vi "Module Loop.vi"(8 "error in (no error)":errorcluster, 11 "Data Processor Module in":refnum<class "Data Processor Module.lvclass">) -> (0 "error out":errorcluster, 3 "Data Processor Module out":refnum<class "Data Processor Module.lvclass">)   [LabVIEW 2020, in "VolatusData.lvlib" / "Data Processor Module.lvclass"]
uses:
  Data Processor Module.lvclass
  C:/dev/lv20CE/relink/lv-volatus/Volatus/Module/Module.lvclass
  Volatus/Module/Module.lvclass
  Data Processor Module.lvclass/Data Processor Module.ctl
  New Data.ctl
  Volatus/Module/Module.lvclass/Module.ctl
  <vilib>/Utility/error.llb/Error Cluster From Error Code.vi
  VolatusData.lvlib
panel:
  out "Parent":string
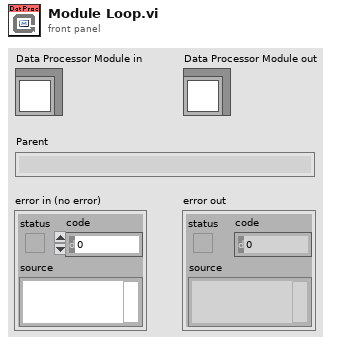
[diagram p1: front panel]
types:
  T1 = enum32{"Invalid", "Standard", "Closed", "Hidden", "Minimized", "Maximized"}
  T2 = typedef "VolatusData.lvlib/New Data.ctl" = cluster{"Channels":waveform(dbl)[]}
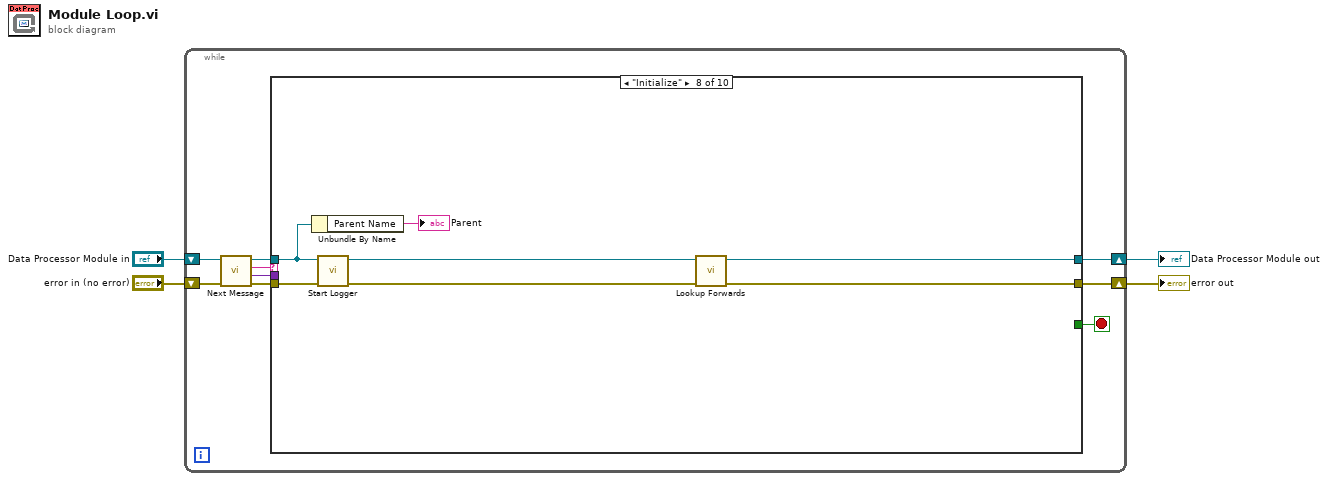
[diagram p0: block diagram]
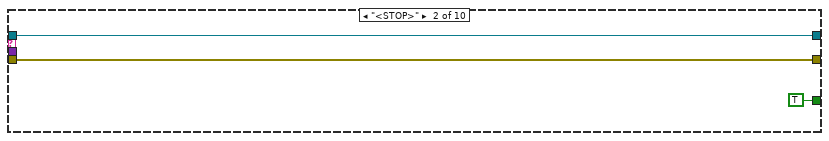
[diagram p3: hidden frame]
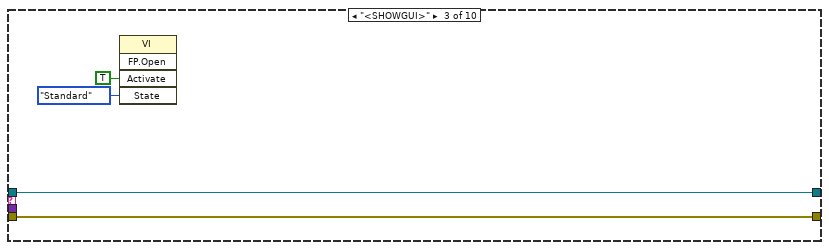
[diagram p4: hidden frame]
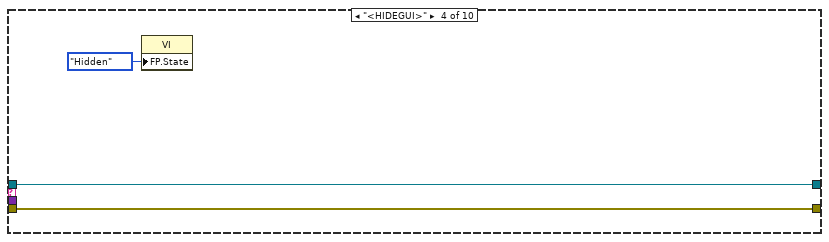
[diagram p5: hidden frame]
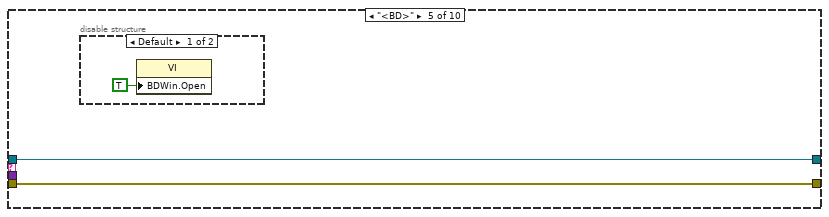
[diagram p6: hidden frame]
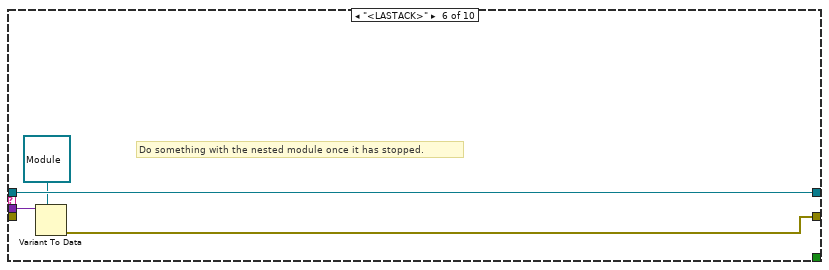
[diagram p8: hidden frame]
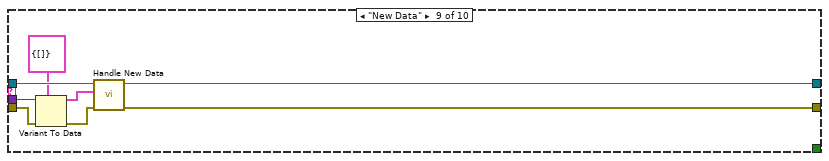
[diagram p10: hidden frame]
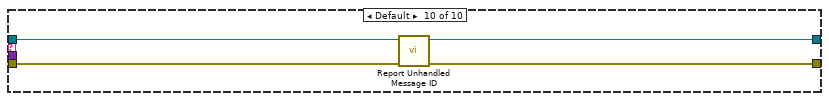
[diagram p11: hidden frame]
diagram:
  n1 = while {
    shift-right: [w8] -> w4
    shift-left: "Data Processor Module in" -> [w13]
    shift-right: [w7] -> w3
    shift-left: "error in (no error)" -> [w12]
    stop <- w6 stop-if-true
    n2 = call "Next Message.vi"("error in (no error)"=w12, "Module in"=w13) -> ("error out"=w11:errorcluster, "Data"=w5:variant, "ID"=w10:string, "Module out"=w9:refnum<class "Data Processor Module.lvclass">)  [unwired: 6 in]
    n3 = case shown="\"Initialize\"" w10 {
      tunnel: w11 -> [w14 w17 w21 w24 w26 _ w33 w41 w47 w53]
      tunnel: w9 -> [w15 w18 w22 w25 w27 w32 w34 w39 w49 w51]
      tunnel: [w15 w18 w22 w25 w27 w32 w34 w35 w45 w50] -> w8
      tunnel: [w14 w17 w21 w24 w26 w29 w33 w37 w42 w52] -> w7
      tunnel: [_ TRUE _ _ _ _ _ _ _ _] -> w6
      tunnel: w5 -> [_ _ _ _ _ w31 _ _ w48 _]
      frame "<CLOSE>" {
      }
      frame "<STOP>" {
      }
      frame "<SHOWGUI>" {
        n4 = invoke class="VI" method="FP.Open"("Activate"=TRUE ("Activate?"), "State"=T1."Standard") -> ()  [unwired: 3 in, 5 out]
      }
      frame "<HIDEGUI>" {
        n5 = property class="VI"("FP.State"=T1."Hidden" ("Front Panel Window:State")) -> ()  [unwired: 2 in, 2 out]
      }
      frame "<BD>" {
        n6 = disable-structure shown="Default" {
          frame condition #0 (active) {
            n7 = property class="VI"("BDWin.Open"=TRUE ("Block Diagram Window:Open")) -> ()  [unwired: 2 in, 2 out]
          }
          frame condition #1 {
          }
        }
      }
      frame "<LASTACK>" {
        # "Do something with the nested module once it has stopped."
        n8 = Variant To Data(type=refnum<class "Module.lvclass"> refnum ("Volatus:Module"), Variant=w31) -> (error out=w29:errorcluster)  [unwired: 1 in, 1 out]
      }
      frame "<TIMEOUT>" {
        # "No message for this module was received in time"
      }
      frame "Initialize" {
        n9 = Unbundle By Name(w39) -> ("Parent Name"=→"Parent":string)
        n10 = call "Start Logger.vi"("error in (no error)"=w41, "Data Processor Module in"=w39) -> ("error out"=w40:errorcluster, "Data Processor Module out"=w36:refnum<class "Data Processor Module.lvclass">)  [unwired: 8 in]
        n11 = call "Lookup Forwards.vi"("error in (no error)"=w40, "Data Processor Module in"=w36) -> ("error out"=w37:errorcluster, "Data Processor Module out"=w35:refnum<class "Data Processor Module.lvclass">)  [unwired: 8 in]
      }
      frame "New Data" {
        n12 = Variant To Data(error in=w47, type=T2 {"Channels"=[]} ("New Data"), Variant=w48) -> (data=w44:T2, error out=w43:errorcluster)
        n13 = call "Handle New Data.vi"("error in (no error)"=w43, "New Data"=w44, "Data Processor Module in"=w49) -> ("error out"=w42:errorcluster, "Data Processor Module out"=w45:refnum<class "Data Processor Module.lvclass">)  [unwired: 7 in]
      }
      frame Default {
        n14 = call "Report Unhandled Message ID.vi"("error in (no error)"=w53, "Module in"=w51) -> ("error out"=w52:errorcluster, "Module out"=w50:refnum<class "Data Processor Module.lvclass">)  [unwired: 8 in]
      }
    }
  }
  "error out" <- w3
  "Data Processor Module out" <- w4
